vi "Main.vi"(9 "B":dbl, 11 "A":dbl) -> (3 "x+y":dbl)   [LabVIEW 2025]
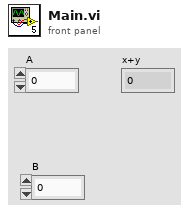
[diagram p1: front panel]
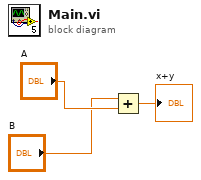
[diagram p0: block diagram]
diagram:
  n1 = Add(x="B", y="A") -> (x+y=→"x+y":dbl)
